vi "PeriodicFilter-Check Speed.vi"(7 "Seconds Since 1Jan1904":timestamp, 8 "Settings":T3={"threashold(#/s)"=1.0, "Check Peroid(s)"=1.0}, 9 "Parameter":string, 10 "Index":i32, 11 "Data In":T1 {"LastCheckT" format="%<%.3X>T"}) -> (0 "Over Threshold?":bool, 1 "New Filtered Item":bool, 3 "Data Out":T1 {"LastCheckT" format="%<%.3X>T"})   [LabVIEW 2017, in "Communicable State Machine.lvlib"]
uses:
  Communicable State Machine.lvlib
  Periodic String Filter Setting.ctl
  Periodic String Filter Data.ctl
  Periodic String Filter Info.ctl
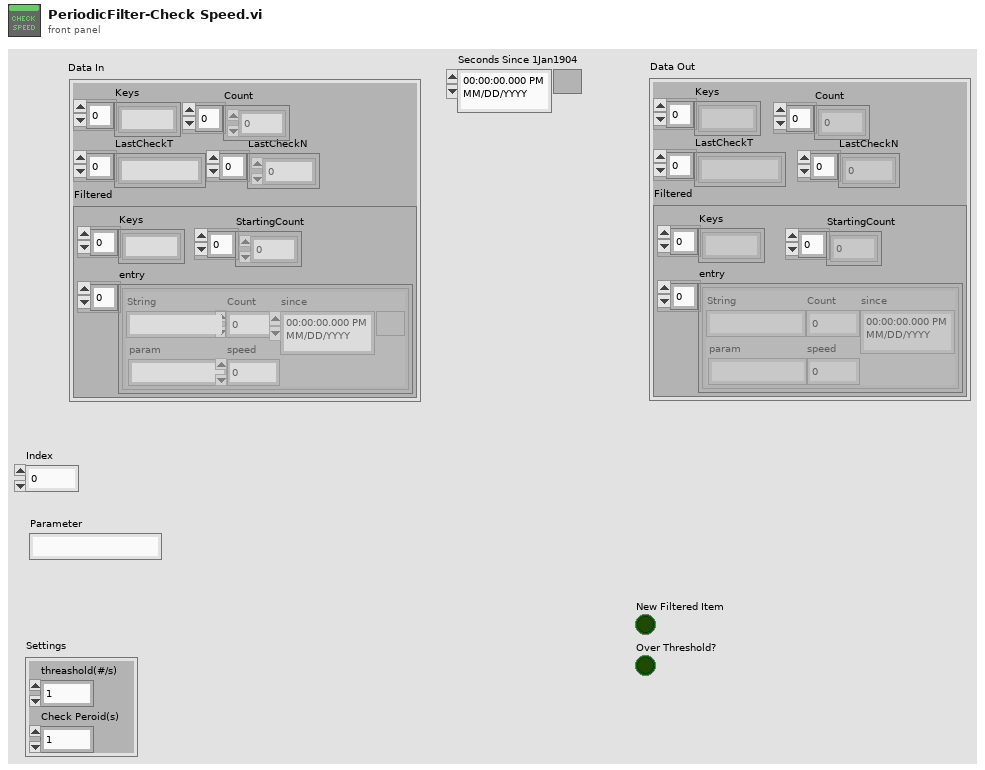
[diagram p1: front panel]
types:
  T1 = typedef "Communicable State Machine.lvlib/Periodic String Filter Data.ctl" = cluster{"Keys":string[], "Count":i64[], "LastCheckT":timestamp[], "LastCheckN":i64[], "Filtered":cluster{"Keys":string[], "StartingCount":i64[], "entry":T2[]}}
  T2 = typedef "Communicable State Machine.lvlib/Periodic String Filter Info.ctl" = cluster{"String":string, "Count":i64, "since":timestamp, "param":string, "speed":dbl}
  T3 = typedef "Communicable State Machine.lvlib/Periodic String Filter Setting.ctl" = cluster{"threashold(#/s)":dbl, "Check Peroid(s)":dbl}
  T4 = cluster{"Keys":string[], "StartingCount":i64[], "entry":T2[]}
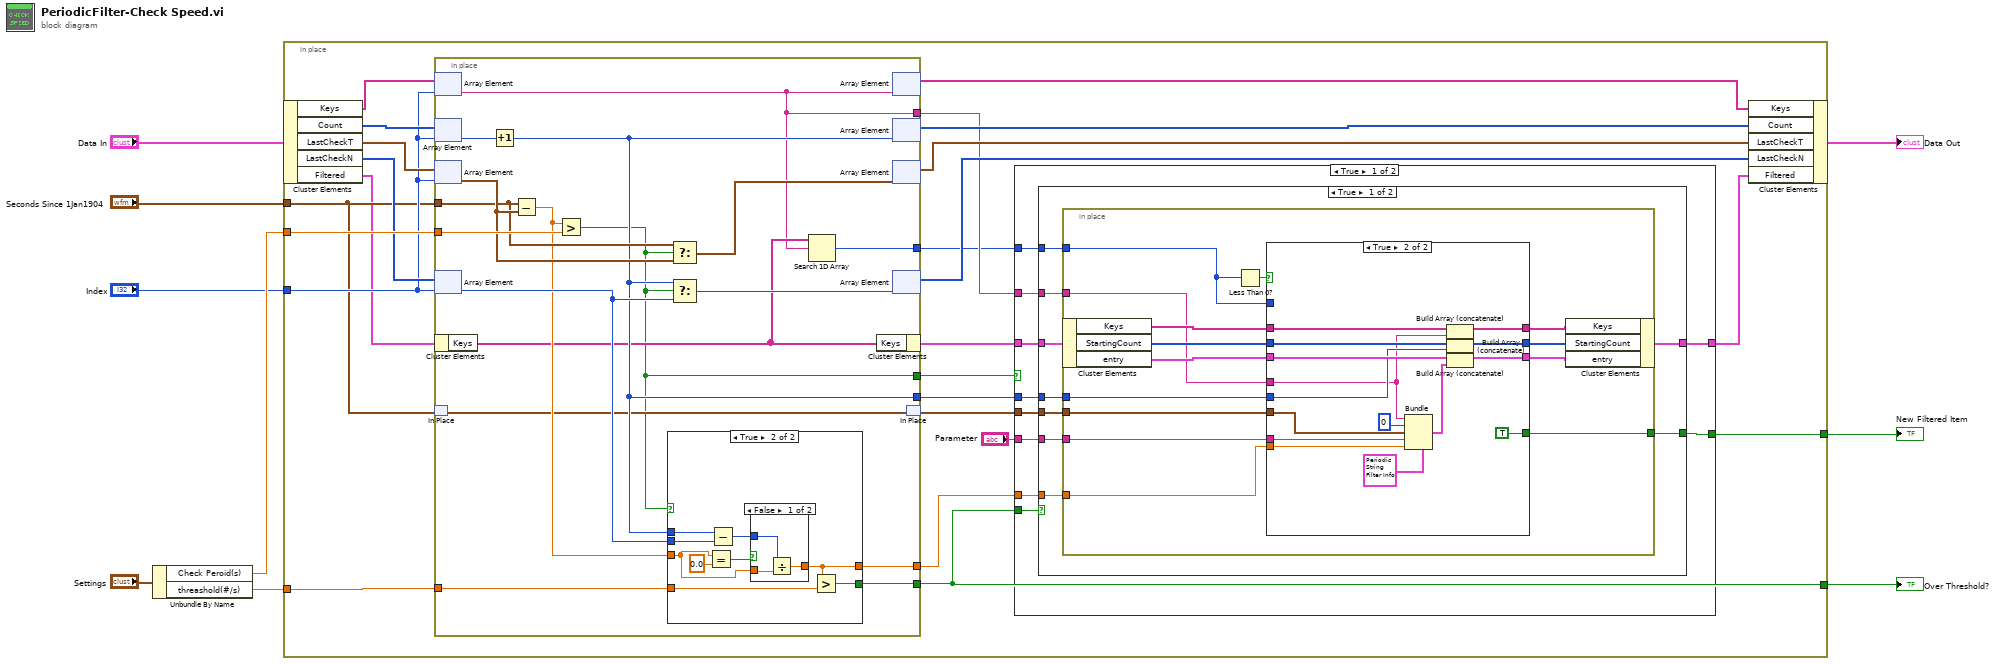
[diagram p0: block diagram]
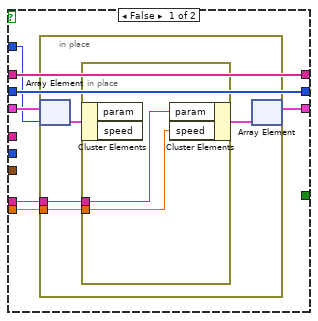
[diagram p2: hidden frame]
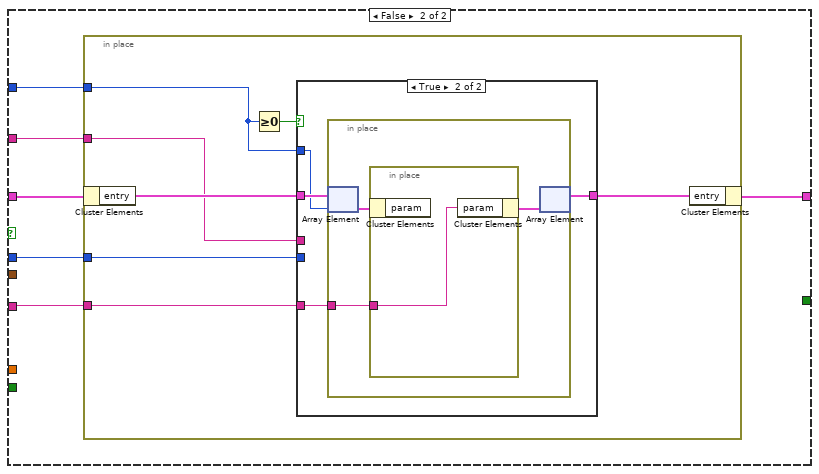
[diagram p4: hidden frame]
diagram:
  n1 = Unbundle By Name("Settings") -> ("Check Peroid(s)"=w9:dbl, "threashold(#/s)"=w8:dbl)
  n2 = in-place "In Place Element Structure" {
    in-place-border: w9 -> [w33]
    in-place-border: "Index" -> [w24]
    in-place-border: w8 -> [w32]
    in-place-border: [w19] -> w6
    in-place-border: "Seconds Since 1Jan1904" -> [w17]
    in-place-border: [w18] -> w1
    n3 = in-place-cluster #1("Data In") -> ("Keys"=w25:string[], "Count"=w31:i64[], "LastCheckT"=w28:timestamp[], "LastCheckN"=w29:i64[], "Filtered"=w14:T4)
    n4 = in-place {
      in-place-border: w17 -> [w131]
      in-place-border: w33 -> [w133]
      in-place-border: w32 -> [w127]
      in-place-border: [w126] -> w19
      in-place-border: [w125] -> w20
      in-place-border: [w120] -> w23
      in-place-border: [w122] -> w15
      in-place-border: [w119] -> w12
      in-place-border: [w118] -> w10
      n5 = in-place-array #2(w25, w24) -> (w120:string)
      n6 = in-place-array #3(w31, w24) -> (w134:i64)
      n7 = in-place-array #4(w28, w24) -> (w132:timestamp)
      n8 = in-place-array #5(w29, w24) -> (w128:i64)
      n9 = in-place-cluster #6(w14) -> ("Keys"=w121:string[])
      n10 = in-place-match #7(w17) -> (w123:timestamp)
      n11 = Increment(x=w134) -> (x+1=w125:i64)
      n12 = Subtract(x=w131, y=w132) -> (x-y=w124:dbl)
      n13 = Greater?(x=w124, y=w133) -> (0:w118:bool)
      n14 = case shown="True" w118 {
        tunnel: w128 -> [_ w142]
        tunnel: w127 -> [_ w141]
        tunnel: [_ w140] -> w126
        tunnel: w125 -> [_ w139]
        tunnel: w124 -> [_ w138]
        tunnel: [_ w135] -> w122
        frame False {
        }
        frame True {
          n15 = Equal?(x=w138, y=0.0) -> (x = y?=w136:bool)
          n16 = Subtract(x=w139, y=w142) -> (x-y=w143:i64)
          n17 = case shown="False" w136 {
            tunnel: [w146 _] -> w135
            tunnel: w143 -> [w145 _]
            tunnel: w138 -> [w144 _]
            frame False {
              n18 = Divide(x=w145, y=w144) -> (x/y=w146:dbl)
            }
            frame True {
            }
          }
          n19 = Greater?(x=w135, y=w141) -> (0:w140:bool)
        }
      }
      n20 = Select(t=w131, s=w118, f=w132) -> (s? t:f=w129:timestamp)
      n21 = Select(t=w125, s=w118, f=w128) -> (s? t:f=w130:i64)
      n22 = Search 1D Array(1D array=w121, element=w120) -> (index of element=w119:i32)  [unwired: 1 in]
      n23 = in-place-cluster #6("Keys"=w121) -> (w13:T4)
      n24 = in-place-array #2(w120) -> (w21:string[])  [unwired: 1 out]
      n25 = in-place-array #3(w125) -> (w30:i64[])  [unwired: 1 out]
      n26 = in-place-array #4(w129) -> (w27:timestamp[])  [unwired: 1 out]
      n27 = in-place-array #5(w130) -> (w26:i64[])  [unwired: 1 out]
      n28 = in-place-match #7(w123) -> (w16:timestamp)
    }
    n29 = case shown="True" w10 {
      tunnel: w23 -> [w43 w101]
      tunnel: [w42 w100] -> w22
      tunnel: w20 -> [w41 w99]
      tunnel: w19 -> [w40 _]
      tunnel: [w39 _] -> w18
      tunnel: w16 -> [w38 _]
      tunnel: w15 -> [w37 _]
      tunnel: w13 -> [w36 w98]
      tunnel: w12 -> [w35 w97]
      tunnel: "Parameter" -> [w34 w96]
      frame True {
        n30 = case shown="True" w40 {
          tunnel: w36 -> [w52 w95]
          tunnel: w38 -> [w51 _]
          tunnel: w43 -> [w50 _]
          tunnel: [w49 w95] -> w42
          tunnel: w41 -> [w48 _]
          tunnel: [w47 _] -> w39
          tunnel: w37 -> [w46 _]
          tunnel: w35 -> [w45 _]
          tunnel: w34 -> [w44 _]
          frame True {
            n31 = in-place {
              in-place-border: w51 -> [w59]
              in-place-border: w50 -> [w58]
              in-place-border: w48 -> [w57]
              in-place-border: [w56] -> w47
              in-place-border: w46 -> [w55]
              in-place-border: w45 -> [w54]
              in-place-border: w44 -> [w53]
              n32 = in-place-cluster #8(w52) -> ("Keys"=w65:string[], "StartingCount"=w63:i64[], "entry"=w64:T2[])
              n33 = Less Than 0?(x=w54) -> (x < 0?=w66:bool)
              n34 = case shown="True" w66 {
                tunnel: w65 -> [w73 w93]
                tunnel: w58 -> [_ w87]
                tunnel: [w73 w94] -> w62
                tunnel: w54 -> [w69 _]
                tunnel: w63 -> [w72 w92]
                tunnel: [w72 w91] -> w61
                tunnel: w64 -> [w71 w90]
                tunnel: w59 -> [_ w86]
                tunnel: [w70 w89] -> w60
                tunnel: w57 -> [_ w88]
                tunnel: [_ TRUE] -> w56
                tunnel: w53 -> [w68 w82]
                tunnel: w55 -> [w67 w80]
                frame False {
                  n35 = in-place {
                    in-place-border: w68 -> [w75]
                    in-place-border: w67 -> [w74]
                    n36 = in-place-array #9(w71, w69) -> (w77:T2)
                    n37 = in-place {
                      in-place-border: w75 -> [w79]
                      in-place-border: w74 -> [w78]
                      n38 = in-place-cluster #10(w77) -> ()  [unwired: 2 out]
                      n39 = in-place-cluster #10("param"=w79, "speed"=w78) -> (w76:T2)
                    }
                    n40 = in-place-array #9(w76) -> (w70:T2[])  [unwired: 1 out]
                  }
                }
                frame True {
                  n41 = Bundle(cluster=T2 {"String"="", "Count"=0, "since"=timestamp(0 s since 1904-01-01), "param"="", "speed"=0.0}, "String"=w87, "Count"=i64 0, "since"=w86, "param"=w82, "speed"=w80) -> (w84:T2)
                  n42 = Build Array (concatenate)(w93, w87) -> (w94:string[])
                  n43 = Build Array (concatenate)(w92, w88) -> (w91:i64[])
                  n44 = Build Array (concatenate)(w90, w84) -> (w89:T2[])
                }
              }
              n45 = in-place-cluster #8("Keys"=w62, "StartingCount"=w61, "entry"=w60) -> (w49:T4)
            }
          }
          frame False {
          }
        }
      }
      frame False {
        n46 = in-place {
          in-place-border: w101 -> [w106]
          in-place-border: w99 -> [w105]
          in-place-border: w96 -> [w104]
          in-place-border: w97 -> [w102]
          n47 = in-place-cluster #11(w98) -> ("entry"=w108:T2[])
          n48 = Greater Or Equal To 0?(x=w102) -> (x >= 0?=w103:bool)
          n49 = case shown="True" w103 {
            tunnel: w106 -> [_ _]
            tunnel: w102 -> [_ w111]
            tunnel: w108 -> [w109 w113]
            tunnel: [w109 w112] -> w107
            tunnel: w105 -> [_ _]
            tunnel: w104 -> [_ w110]
            frame False {
            }
            frame True {
              n50 = in-place {
                in-place-border: w110 -> [w114]
                n51 = in-place-array #12(w113, w111) -> (w116:T2)
                n52 = in-place {
                  in-place-border: w114 -> [w117]
                  n53 = in-place-cluster #13(w116) -> ()  [unwired: 1 out]
                  n54 = in-place-cluster #13("param"=w117) -> (w115:T2)
                }
                n55 = in-place-array #12(w115) -> (w112:T2[])  [unwired: 1 out]
              }
            }
          }
          n56 = in-place-cluster #11("entry"=w107) -> (w100:T4)
        }
      }
    }
    n57 = in-place-cluster #1("Keys"=w21, "Count"=w30, "LastCheckT"=w27, "LastCheckN"=w26, "Filtered"=w22) -> (→"Data Out":T1)
  }
  "Over Threshold?" <- w6
  "New Filtered Item" <- w1
